vi "PicoScope5000aExampleAWG.vi"() -> ()   [LabVIEW 2010]
uses:
  ps5000a.dll
panel:
  out "error out":errorcluster
  out "USB 3.0 device on non-USB 3.0 Port":bool=TRUE
  out "USB Powered":bool=TRUE
  in  "Arbitrary Waveform Settings":T1 {"Index Mode" items=["Single", "Dual", "Quad"]}
  in  "General AWG Settings":T2={"Peak-to-Peak Voltage (microvolts)"=2000000, "Offset Voltage (microvolts)"=0, "Wave Type"=0, "Sweep Type"=0, "Shots"=0, "Sweeps"=0, "Trigger Type"=0, "Trigger Source"=0, "Ext. Threshold (ADC count)"=0, "White Noise/PRBS"=0} {"White Noise/PRBS" items=["Normal", "White Noise", "PRBS"]; "Trigger Source" items=["None", "Scope Trigger", "Aux. In", "Ext. In", "Software Trigger"]; "Trigger Type" items=["Rising", "Falling", "Gate High", "Gate Low"]; "Sweep Type" items=["Up", "Down", "Up-Down", "Down-Up"]; "Wave Type" items=["Sine", "Square", "Triangle", "Ramp Up", "Ramp Down", "Sinc", "Gaussian", "Half Sine", "DC", "Arbitrary"]}
  in  "Standard Waveform Settings":T3={"Start Frequency"=1000.0, "Stop Frequency"=1000.0, "Increment"=0.0, "Dwell Time (seconds)"=0.0} {"Stop Frequency" min=0.03 max=1000000.0; "Start Frequency" min=0.03 max=1000000.0}
  in  "Serial Number":string
  in  "Open using Serial Number":bool
  in  "Scope Resolution":u32(ring) items=["8-bit", "12-bit", "14-bit", "15-bit", "16-bit"]
  in  "Stop S/W \nTrigger":bool
  in  "Apply Settings":bool
  in  "Stop VI":bool
  in  "Software \nTrigger":bool
  out "Arbitrary\nWaveform Graph":i16[](graph)
  # "If Software trigger is selected, press the 'Stop S/W Trigger'\nbutton prior to selecting 'Apply Settings' or 'Stop VI'."
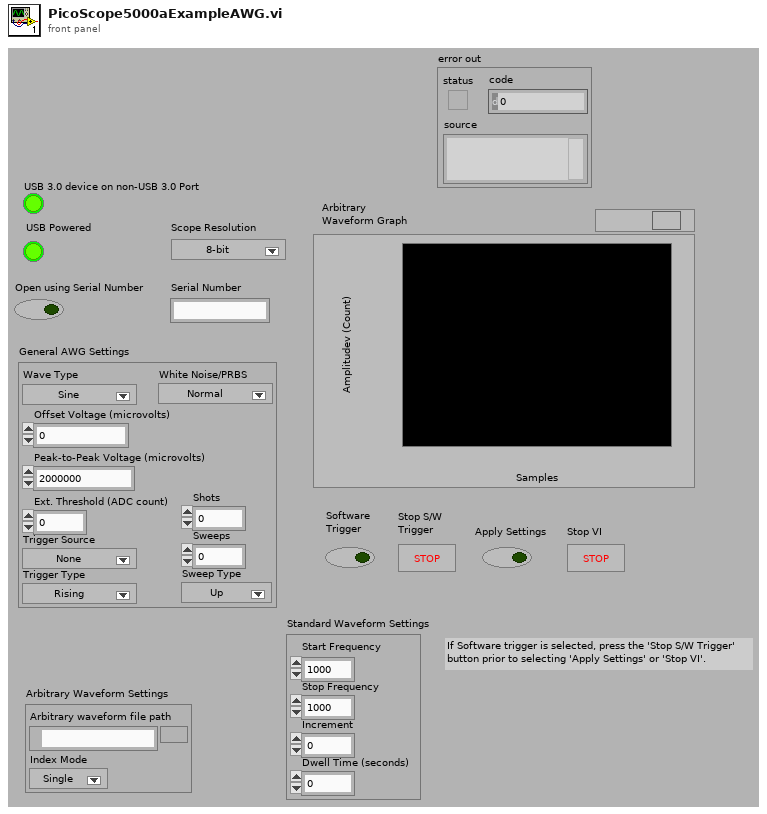
[diagram p1: front panel]
types:
  T1 = cluster{"Arbirary waveform file path":path, "Index Mode":u32}
  T2 = cluster{"Peak-to-Peak Voltage (microvolts)":u32, "Offset Voltage (microvolts)":i32, "Wave Type":u32, "Sweep Type":u32, "Shots":u32, "Sweeps":u32, "Trigger Type":u32, "Trigger Source":u32, "Ext. Threshold (ADC count)":i16, "White Noise/PRBS":u32}
  T3 = cluster{"Start Frequency":dbl, "Stop Frequency":dbl, "Increment":dbl, "Dwell Time (seconds)":dbl}
  T4 = cluster{"status":bool, "code":u32, "source":string}
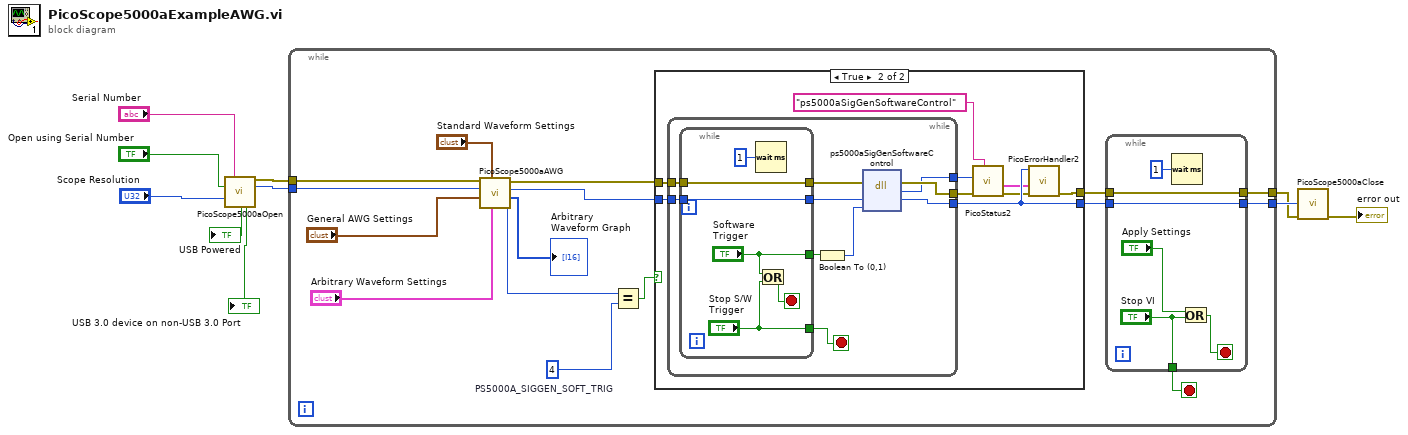
[diagram p0: block diagram]
diagram:
  n1 = call "PicoScope5000aOpen.vi"("Serial Number"="Serial Number", "Use Serial Number"="Open using Serial Number", "Resolution"="Scope Resolution") -> ("USB 3.0 device on non-USB 3.0 Port"=→"USB 3.0 device on non-USB 3.0 Port":bool, "error out"=w9:errorcluster, "handle"=w10:i16, "USB Powered"=→"USB Powered":bool)  [unwired: 7 in, 2 out]
  n2 = while {
    tunnel: w10 -> [w25]
    tunnel: w9 -> [w24]
    tunnel: [w18] -> w8
    tunnel: [w12] -> w2
    stop <- w17 stop-if-true
    w23 = 4  # PS5000A_SIGGEN_SOFT_TRIG
    n3 = call "PicoScope5000aAWG.vi"("Arbitrary Waveform Settings"="Arbitrary Waveform Settings", "Standard Waveform Settings"="Standard Waveform Settings", "General AWG Settings"="General AWG Settings", "Handle In"=w25, "error in"=w24) -> ("Trigger Source Out"=w19:u32, "Arbitrary\nWaveform Graph"=→"Arbitrary\nWaveform Graph":i16[], "Handle Out"=w20:i16, "error out"=w21:errorcluster)  [unwired: 3 in]
    n4 = Equal?(x=w19, y=w23) -> (x = y?=w22:bool)
    n5 = case shown="True" w22 {
      tunnel: w21 -> [w33 w43]
      tunnel: [w34 w41] -> w13
      tunnel: w20 -> [w34 w42]
      tunnel: [w33 w40] -> w11
      frame False {
      }
      frame True {
        n6 = while {
          tunnel: w43 -> [w52]
          tunnel: w42 -> [w51]
          tunnel: [w49] -> w41
          tunnel: [w45] -> w39
          tunnel: [w44] -> w38
          stop <- w46 stop-if-true
          n7 = while {
            tunnel: [w59] -> w53
            tunnel: w52 -> [w59]
            tunnel: ["Software \nTrigger"] -> w48
            tunnel: w51 -> [w58]
            tunnel: [w58] -> w50
            tunnel: ["Stop S/W \nTrigger"] -> w46
            stop <- w55 stop-if-true
            n8 = Wait (ms)(milliseconds to wait=u32 1) -> ()  [unwired: 1 out]
            n9 = Or(x="Software \nTrigger", y="Stop S/W \nTrigger") -> (x .or. y?=w55:bool)
          }
          n10 = Boolean To (0,1)(Boolean=w48) -> (0, 1=w47:i16)
          n11 = dll-call lib="ps5000a.dll" fn="ps5000aSigGenSoftwareControl"(error in=w53, "handle"=w50, "state"=w47) -> (error out=w45:errorcluster, "PICO_STATUS"=w44:u32, "handle"=w49:i16)  [unwired: 3 in, 1 out]
        }
        n12 = call "PicoStatus2.vi"("PICO source"="ps5000aSigGenSoftwareControl" ("source"), "Error in"=w39, "PICO STATUS"=w38) -> ("error out"=w37:errorcluster, "PICO_STATUS out"=w35:T4)  [unwired: 5 in]
        n13 = call "PicoErrorHandler2.vi"("error in (no error)"=w37, "PICO_STATUS in"=w35, "handle In"=w41) -> ("error out"=w40:errorcluster)  [unwired: 8 in]
      }
    }
    n14 = while {
      tunnel: ["Stop VI"] -> w17
      tunnel: [w32] -> w18
      tunnel: w13 -> [w32]
      tunnel: [w28] -> w12
      tunnel: w11 -> [w28]
      stop <- w31 stop-if-true
      n15 = Wait (ms)(milliseconds to wait=u32 1) -> ()  [unwired: 1 out]
      n16 = Or(x="Apply Settings", y="Stop VI") -> (x .or. y?=w31:bool)
    }
  }
  n17 = call "PicoScope5000aClose.vi"("error in (no error)"=w2, "handle in"=w8) -> ("error out"=→"error out":errorcluster)  [unwired: 8 in, 1 out]
